vi "Initialize Tree.vi"(8 "error in":errorcluster, 11 "Module Data":T1={"PeekVI Reference"=refnum, "SubPanel"=refnum, "Peek Stack Tree Ref"=refnum, "Open Button Ref"=refnum, "Top VI"=refnum, "Active VI"=refnum, "Stack"=[], "Last FP State"=enum."Standard"}) -> (0 "error out":errorcluster, 3 "Module Data":T1={"PeekVI Reference"=refnum, "SubPanel"=refnum, "Peek Stack Tree Ref"=refnum, "Open Button Ref"=refnum, "Top VI"=refnum, "Active VI"=refnum, "Stack"=[], "Last FP State"=enum."Standard"})   [LabVIEW 2020, in "Peek Window.lvlib"]
uses:
  Peek Window.lvlib
  MHL Data Cluster.ctl
  VI Types/Standard VI Type/Standard VI Type.lvclass
  Symbols Enum.ctl
  cb685dd4-87ab-4bc3-90dd-f8513bb521dc.vi
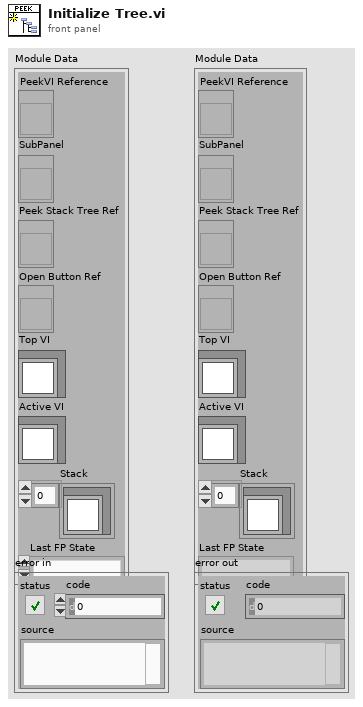
[diagram p1: front panel]
types:
  T1 = typedef "Peek Window.lvlib/MHL Data Cluster.ctl" = cluster{"PeekVI Reference":refnum<vi>, "SubPanel":refnum<vi>, "Peek Stack Tree Ref":refnum<vi>, "Open Button Ref":refnum<vi>, "Top VI":refnum<class "Standard VI Type.lvclass">, "Active VI":refnum<class "Standard VI Type.lvclass">, "Stack":refnum<class "Standard VI Type.lvclass">[], "Last FP State":enum32{"Invalid", "Standard", "Closed", "Hidden", "Minimized", "Maximized"}}
  T2 = typedef "Peek Window.lvlib/Symbols Enum.ctl" = enum16{"<Blank>", "Implementation Mark", "Standard VI", "Dynamic Dispatch VI", "Malleable VI", "Polymorphic VI", "Missing VI", "Express VI"}
  T3 = typedef "imagedata.ctl" = cluster{"image type":i32, "image depth":i32, "image":u8[], "mask":u8[], "colors":u32[], "Rectangle":cluster{"left":i16, "top":i16, "right":i16, "bottom":i16}}
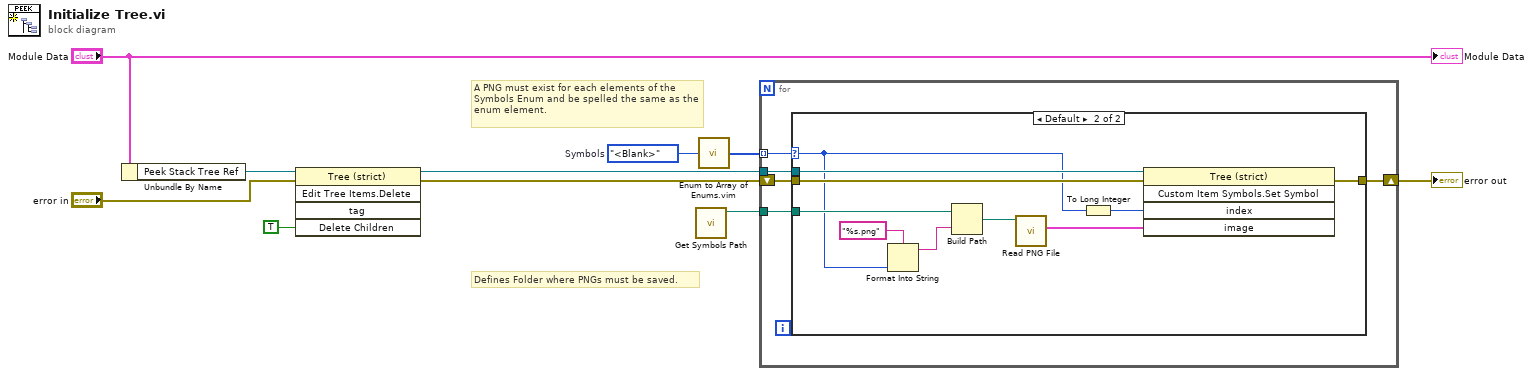
[diagram p0: block diagram]
diagram:
  w3 = Symbols_Enum."<Blank>"  # Symbols
  # "Defines Folder where PNGs must be saved."
  # "A PNG must exist for each elements of the Symbols Enum and be spelled the same as the enum element."
  n1 = Unbundle By Name("Module Data") -> ("Peek Stack Tree Ref"=w10:refnum<vi>)
  n2 = invoke class="Tree (strict)" method="Edit Tree Items.Delete"(reference=w10, error in="error in", "Delete Children"=TRUE ("Delete Children?")) -> (reference out=w8:refnum<vi>, error out=w7:errorcluster)  [unwired: 2 in, 3 out]
  n3 = call "Get Symbols Path.vi"() -> ("path"=w4:path)  [unwired: 11 in]
  n4 = call "Enum to Array of Enums.vim"("enum"=w3) -> ("array of enums"=w1:T2[])
  n5 = for {
    tunnel: w8 -> [w15]
    tunnel: w4 -> [w13]
    shift-right: [w12] -> w2
    shift-left: w7 -> [w14]
    tunnel: w1 -> [w11] mode=indexing
    n6 = case shown="Default" w11 {
      selector: w11 -> [_ w19]
      tunnel: w15 -> [_ w26]
      tunnel: w14 -> [w16 w25]
      tunnel: w13 -> [_ w22]
      tunnel: [w16 w21] -> w12
      frame "<Blank>" {
      }
      frame Default {
        n7 = Format Into String(format string="%s.png", w19) -> (resulting string=w17:string)  [unwired: 2 in, 1 out]
        n8 = Build Path(base path=w22, name or relative path=w17) -> (appended path=w24:path)
        n9 = call <vilib>:"Read PNG File.vi"("path to PNG file"=w24) -> ("image data"=w23:T3)  [unwired: 8 in, 2 out]
        n10 = To Long Integer(number=w19) -> (32bit integer=w20:i32)
        n11 = invoke class="Tree (strict)" method="Custom Item Symbols.Set Symbol"(reference=w26, error in=w25, "index"=w20, "image"=w23) -> (error out=w21:errorcluster)  [unwired: 1 in, 4 out]
      }
    }
  }
  "error out" <- w2
  "Module Data" <- "Module Data"
